vi "W19_ConfigPath.vi"() -> ()   [LabVIEW 2026]
doc: "Use this template to build a VI to use as a subVI."
uses:
  <vilib>/Utility/sysdir.llb/System Directory Type.ctl
panel:
  out "error out":errorcluster
  out "already existed?":bool
  out "config path":path
  # "station_template.ini must sit next to this VI (or the EXE)."
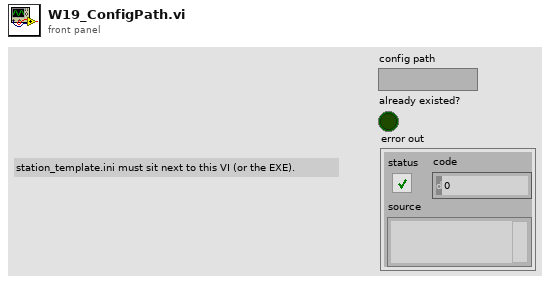
[diagram p1: front panel]
types:
  T1 = typedef "System Directory Type.ctl" = i32
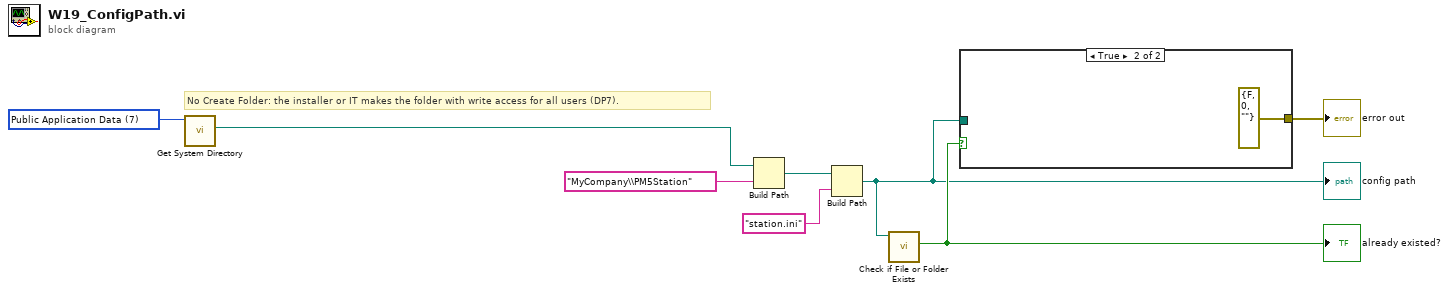
[diagram p0: block diagram]
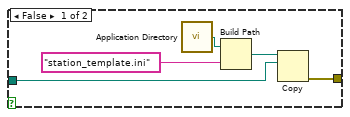
[diagram p2: hidden frame]
diagram:
  w8 = T1 7 items=["User Home"=0, "User Desktop"=1, "User Documents"=2, "User Application Data"=3, "User Preferences"=4, "User Temporary"=5, "Public Documents"=6, "Public Application Data"=7, "Public Preferences"=8, "Public Cache"=13, "System Core Libraries"=9, "System Installed Libraries"=10, "Application Files"=11, "Boot Volume Root"=12] ("system directory type")
  # "No Create Folder: the installer or IT makes the folder with write access for all users (DP7)."
  n1 = call <vilib>:"Get System Directory.vi"("system directory type"=w8) -> ("system directory"=w7:path)  [unwired: 10 in]
  n2 = Build Path(base path=w7, name or relative path="MyCompany\\PM5Station") -> (appended path=w5:path)
  n3 = Build Path(base path=w5, name or relative path="station.ini") -> (appended path=w2:path)
  "config path" <- w2
  n4 = call <vilib>:"Check if File or Folder Exists.vi"("path"=w2) -> ("file or folder exists?"=w3:bool)  [unwired: 8 in, 2 out]
  "already existed?" <- w3
  n5 = case shown="True" w3 {
    tunnel: w2 -> [w10 _]
    tunnel: [w9 errorcluster {"status"=FALSE, "code"=0, "source"=""} ("error in (no error)")] -> w1
    frame False {
      n6 = call <vilib>:"Application Directory.vi"() -> ("Application Directory"=w13:path)
      n7 = Build Path(base path=w13, name or relative path="station_template.ini") -> (appended path=w11:path)
      n8 = Copy(10:w10, 11:w11) -> (0:w9:errorcluster)  [unwired: 3 in, 2 out]
    }
    frame True {
    }
  }
  "error out" <- w1
